vi "RFH-convert-libreVNA.vi"(3 "pre-text":string="libreVNA-", 5 "destionation path":path, 7 "All libreVNA data folder":path, 8 "error in (no error)":errorcluster, 9 "Max Frequency (6G)":dbl=6000000000.0, 10 "Min Frequency  (0.3G)":dbl=300000000.0) -> (0 "error out":errorcluster, 1 "All Good?":bool, 2 "last file":path, 4 "Last Value":T1)   [LabVIEW 2020, in "RFH-Reflection_File_Handler.lvlib"]
doc: "Converts every LibreVNA data folder into averaged common-format files in the destination path, limited to the min and max frequency, and verifies the conversion. Returns the last file, its data and whether all is good."
uses:
  RFH-Reflection_File_Handler.lvlib
  RFH-common_data_format.ctl
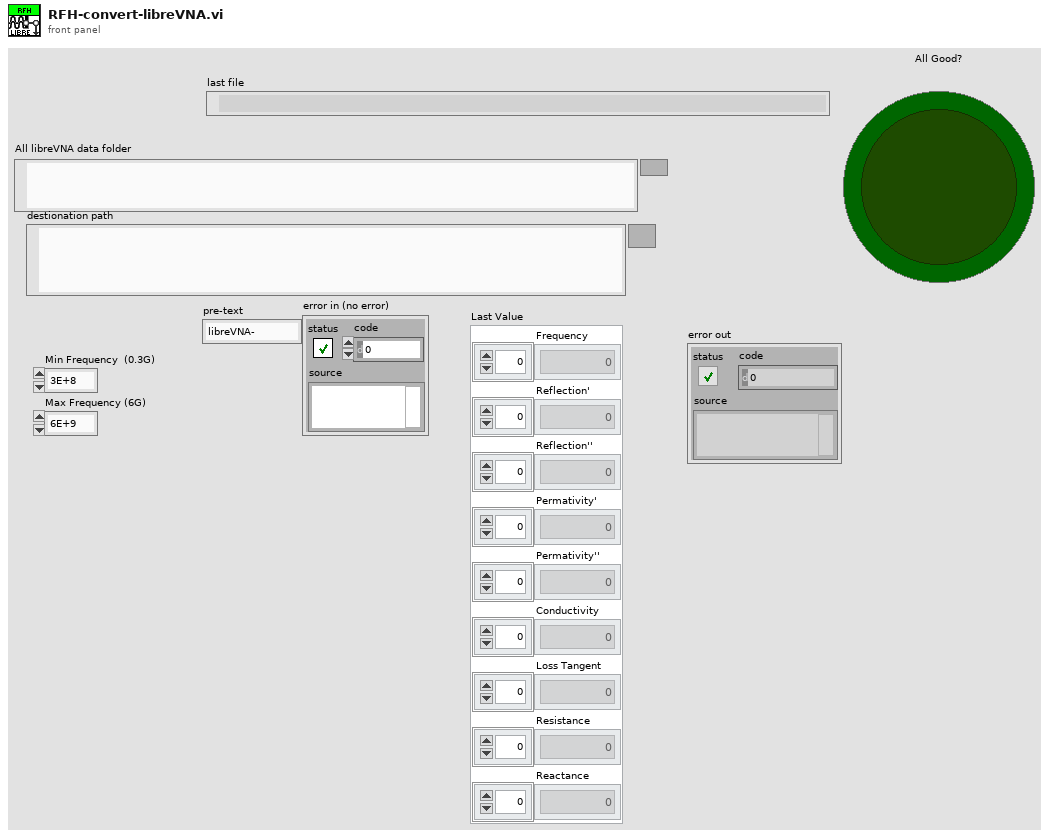
[diagram p1: front panel]
types:
  T1 = typedef "RFH-Reflection_File_Handler.lvlib/RFH-common_data_format.ctl" = cluster{"Frequency":dbl[], "Reflection'":dbl[], "Reflection''":dbl[], "Permativity'":dbl[], "Permativity''":dbl[], "Conductivity":dbl[], "Loss Tangent":dbl[], "Resistance":dbl[], "Reactance":dbl[]}
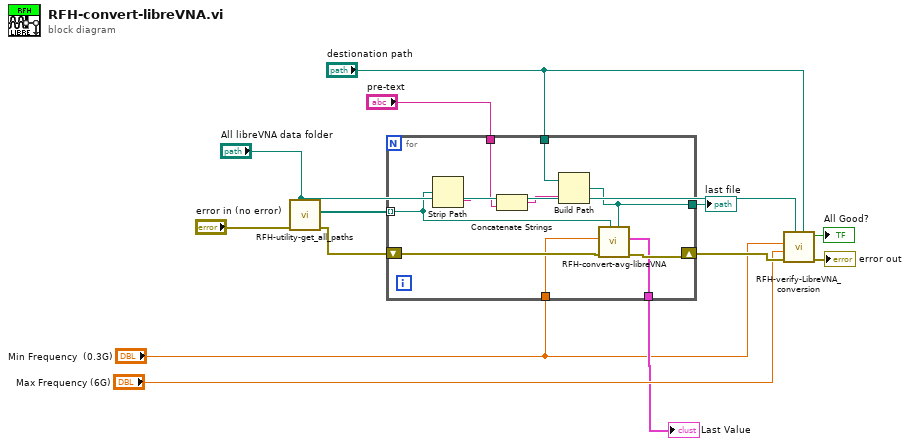
[diagram p0: block diagram]
diagram:
  n1 = call "RFH-utility-get_all_paths.vi"("Folder Path"="All libreVNA data folder", "error in (no error)"="error in (no error)") -> ("error out"=w12:errorcluster, "All Folders"=w13:path[])  [unwired: 6 in, 2 out]
  n2 = for {
    tunnel: w13 -> [w19] mode=indexing
    tunnel: "destionation path" -> [w21]
    shift-right: [w17] -> w6
    shift-left: w12 -> [w20]
    tunnel: [w18] -> w11
    tunnel: [w16] -> w4
    tunnel: "pre-text" -> [w15]
    tunnel: "Min Frequency  (0.3G)" -> [w14]
    n3 = Strip Path(path=w19) -> (name=w22:string)  [unwired: 1 out]
    n4 = Concatenate Strings(w15, w22) -> (w23:string)
    n5 = Build Path(base path=w21, name or relative path=w23) -> (appended path=w18:path)
    n6 = call "RFH-convert-avg-libreVNA.vi"("average filepath"=w18, "Source Folder"=w19, "error in (no error)"=w20, "Frequency low"=w14) -> ("error out"=w17:errorcluster, "Common Format"=w16:T1)  [unwired: 6 in]
  }
  "last file" <- w11
  "Last Value" <- w4
  n7 = call "RFH-verify-LibreVNA_conversion.vi"("Conversion Folder"="destionation path", "Excel File Folder"="All libreVNA data folder", "error in (no error)"=w6, "Max Frequency (6G)"="Max Frequency (6G)", "Min Frequency  (0.3G)"="Min Frequency  (0.3G)") -> ("error out"=→"error out":errorcluster, "All Good?"=→"All Good?":bool)  [unwired: 5 in]
